vi "SMTP Email Send Message Charset.vi"(0 "recipients":string[](array[string]) caption="destinataires", 1 "mail server":string caption="serveur mail", 2 "return address":string caption="adresse de retour", 3 "character set (us-ascii)":string="us-ascii" caption="jeu de caractères (us-ascii)", 5 "subject ([No Subject])":string="[Sans objet]" caption="objet ([Sans objet])", 7 "message":string, 11 "error in (no error)":errorcluster caption="entrée d'erreur (pas d'erreur)", 14 "translit":string="MacRoman iso-8859-1 macroman.trl, ToUpper iso-8859-1 toupper.trl,\nMacRomanUp MacRoman toupper.trl") -> (4 "invalid recipients":string[](array[string]) caption="destinataires non valides", 15 "error out":errorcluster caption="sortie d'erreur")   [LabVIEW 2022 SP3, in "Copie de NI_SMTPEmail.lvlib"]
doc: "Envoie un e-mail texte à une liste de destinataires."
uses:
  Copie de NI_SMTPEmail.lvlib
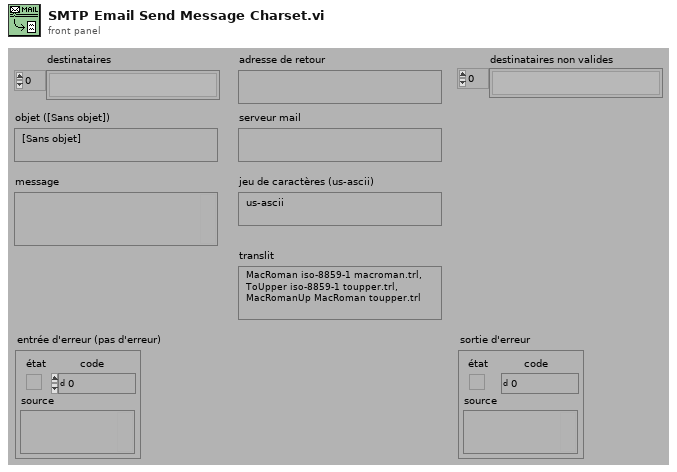
[diagram p1: front panel]
types:
  T1 = typedef "Copie de NI_SMTPEmail.lvlib/SMTP Email Session.ctl" = refnum<k1>
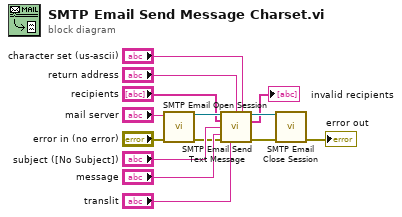
[diagram p0: block diagram]
diagram:
  n1 = call "SMTP Email Open Session.vi"("error in (no error)"="error in (no error)", "mail server"="mail server") -> ("error out"=w2:errorcluster, "smtp session out"=w11:T1)  [unwired: 4 in]
  n2 = call "SMTP Email Send Text Message.vi"("smtp session"=w11, "return address"="return address", "character set"="character set (us-ascii)", "recipients"="recipients", "subject"="subject ([No Subject])", "message"="message", "error in (no error)"=w2, "translit"="translit") -> ("smtp session out"=w9:T1, "invalid recipients"=→"invalid recipients":string[], "error out"=w10:errorcluster)  [unwired: 5 in]
  n3 = call "SMTP Email Close Session.vi"("error in (no error)"=w10, "smtp session"=w9) -> ("error out"=→"error out":errorcluster)  [unwired: 4 in, 1 out]
